vi "Registry.vi"   [LabVIEW 2018, in "GLog.lvlib" / "Registry.lvlib"]
uses:
  Registry.lvlib
  Registry Message.ctl
  Registry Actions.ctl
  api/logger_class/Logger.lvclass
  <vilib>/event_ctls.llb/usereventprio.ctl
  Register Action Data.ctl
  api/logger_class/Logger.lvclass/Logger.ctl
  api/logger_class/Log Record.ctl
  api/logger_class/Internal Log Levels.ctl
  api/logger_class/Log Levels.ctl
  <vilib>/Utility/error.llb/Error Cluster From Error Code.vi
  api/logger_class/Log (Log Record).vi
  <vilib>/ErrorRing/Error Ring.xnode
types:
  T1 = typedef "usereventprio.ctl" = enum32{"high priority", "normal priority"}
  T2 = typedef "GLog.lvlib/Registry.lvlib/Registry Message.ctl" = cluster{"action":T3, "data":variant, "return notifier":refnum<notifier>}
  T3 = typedef "GLog.lvlib/Registry.lvlib/Registry Actions.ctl" = enum16{"Register", "Log", "Enable", "Enable All", "Disable", "Disable All", "Get Enable State", "Get Minimum Log Level", "Set Minimum Log Level", "Set All Minimum Log Level", "Get Logger Info", "Get All Logger Info", "List", "Unregister", "Unregister All", "Shutdown"}
  T4 = typedef "GLog.lvlib/Registry.lvlib/Register Action Data.ctl" = cluster{"Logger":refnum<class "Logger.lvclass">, "Owning VI":string}
  T5 = typedef "GLog.lvlib/Logger.lvclass/Log Record.ctl" = cluster{"level":T6, "timestamp":timestamp, "call chain":string[], "message":string, "data":variant}
  T6 = typedef "GLog.lvlib/Logger.lvclass/Internal Log Levels.ctl" = enum16{"Trace", "Debug", "Info", "Warning", "Error", "Critical", "Internal"}
  T7 = typedef "GLog.lvlib/Logger.lvclass/Log Levels.ctl" = enum16{"Trace", "Debug", "Info", "Warning", "Error", "Critical"}
  T8 = cluster{"logger out":refnum<class "Logger.lvclass">, "error out":errorcluster}
  T9 = cluster{"Enabled?":bool, "error out":errorcluster}
  T10 = cluster{"minimum log level":T7, "error out":errorcluster}
  T11 = cluster{"log level":T7, "error out":errorcluster}
  T12 = cluster{"name":string, "minimum log level":T7, "Enabled?":bool, "error out":errorcluster}
  T13 = cluster{"name":string, "minimum log level":T7, "Enabled?":bool}
  T14 = enum32{"Bad", "Idle", "Run top level", "Running"}[]
  T15 = enum32{"Bad", "Idle", "Run top level", "Running"}
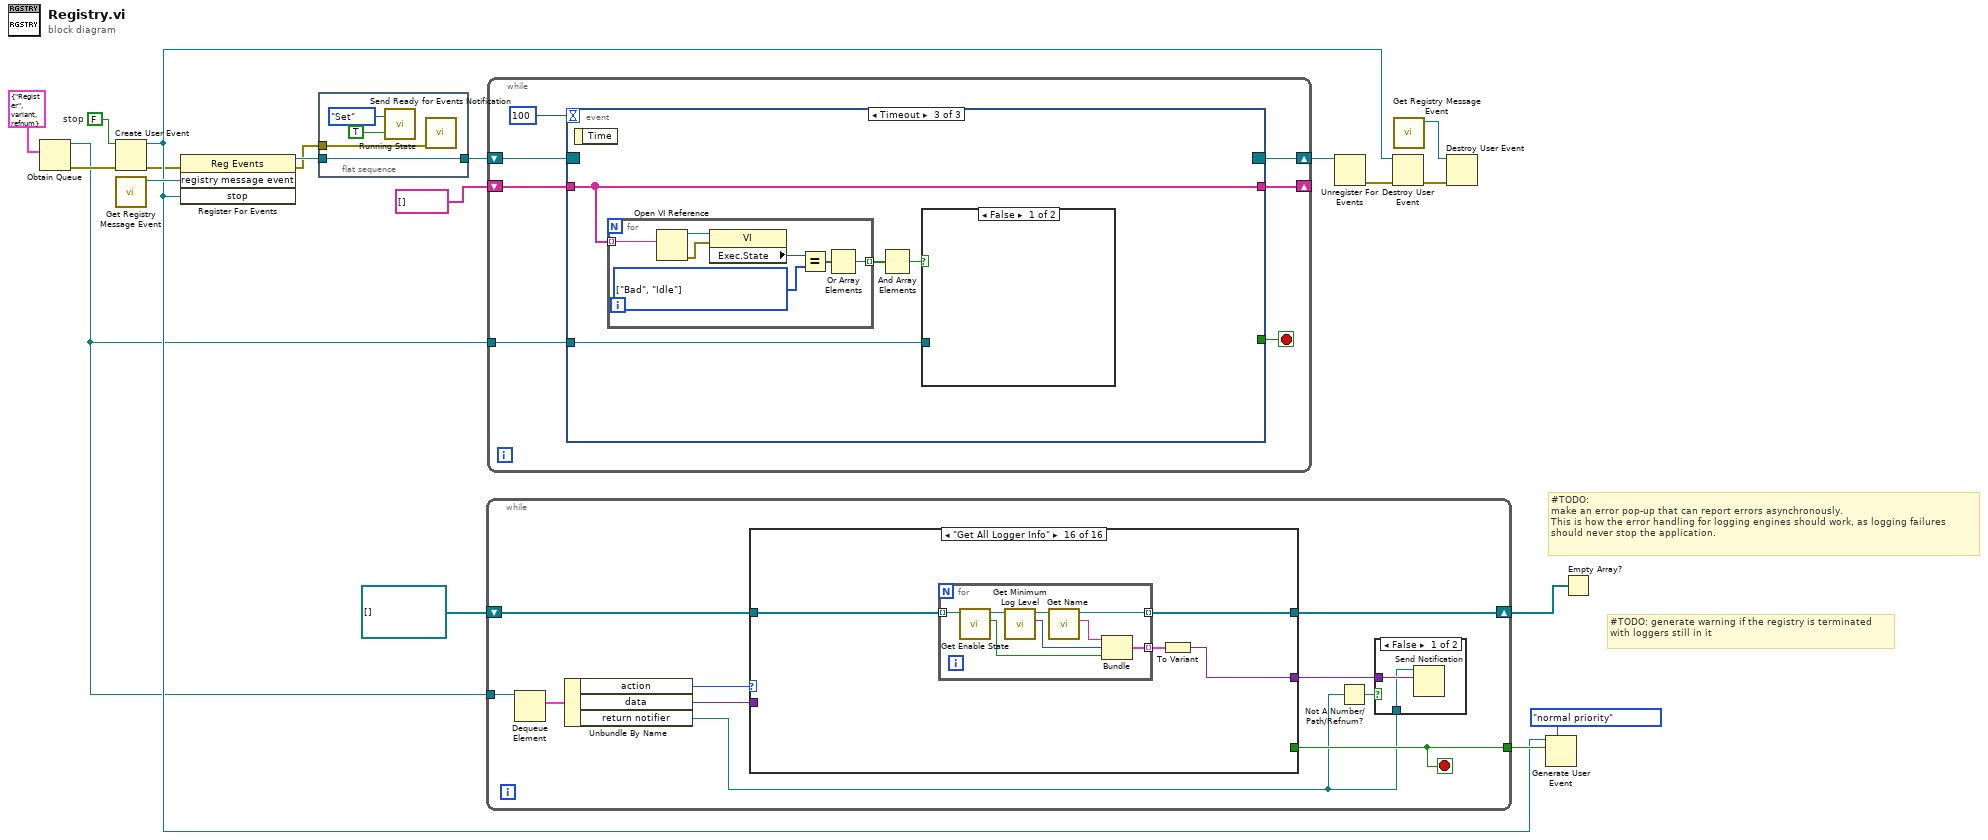
[diagram p0: block diagram]
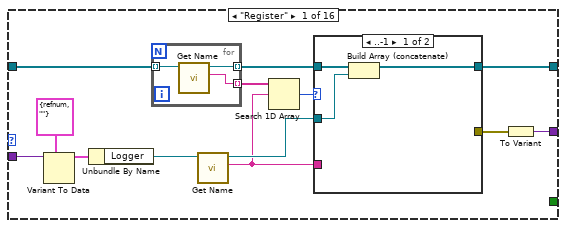
[diagram p2: hidden frame]
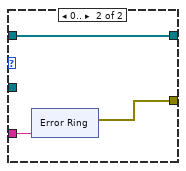
[diagram p3: hidden frame]
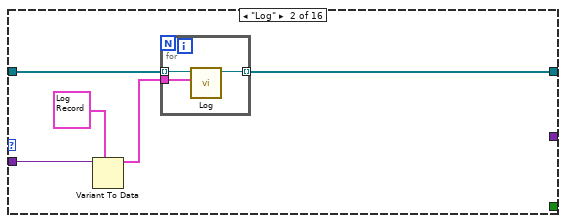
[diagram p4: hidden frame]
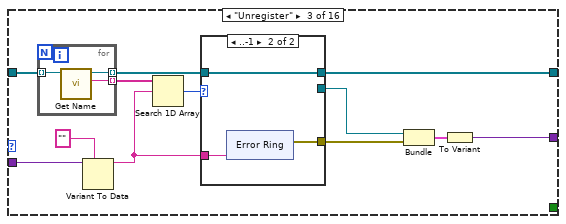
[diagram p5: hidden frame]
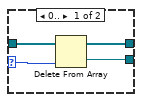
[diagram p6: hidden frame]
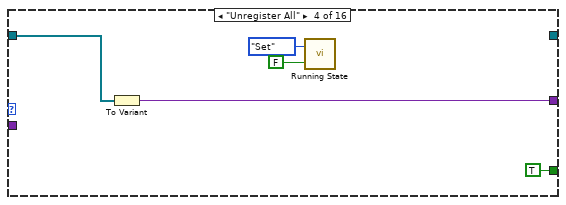
[diagram p7: hidden frame]
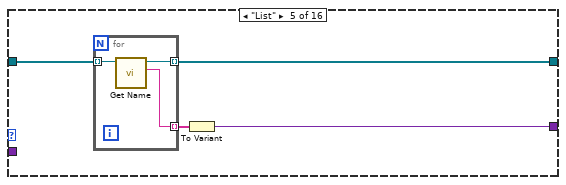
[diagram p8: hidden frame]
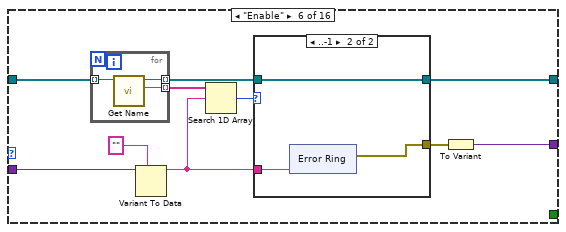
[diagram p9: hidden frame]
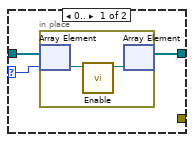
[diagram p10: hidden frame]
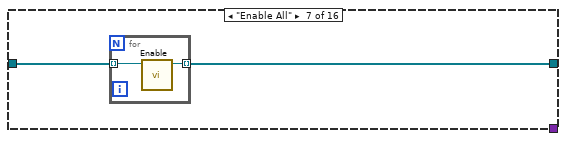
[diagram p11: hidden frame]
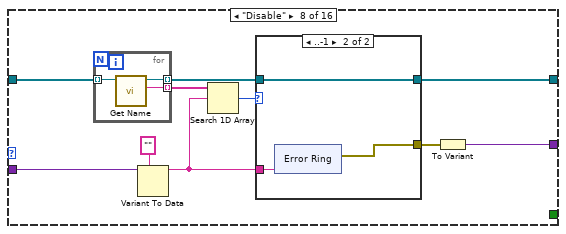
[diagram p12: hidden frame]
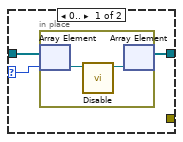
[diagram p13: hidden frame]
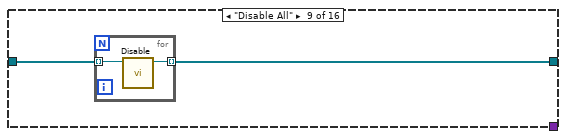
[diagram p14: hidden frame]
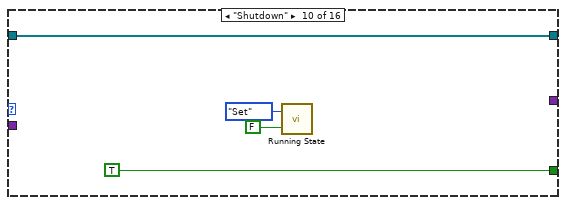
[diagram p15: hidden frame]
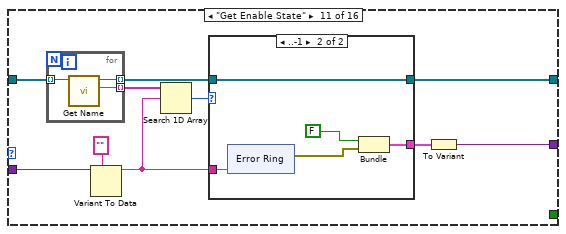
[diagram p16: hidden frame]
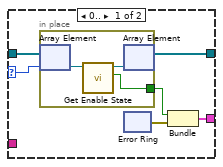
[diagram p17: hidden frame]
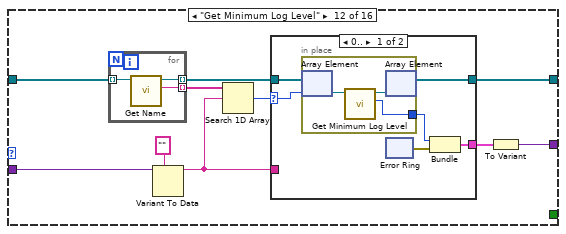
[diagram p18: hidden frame]
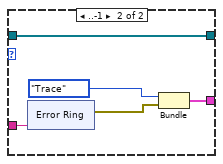
[diagram p19: hidden frame]
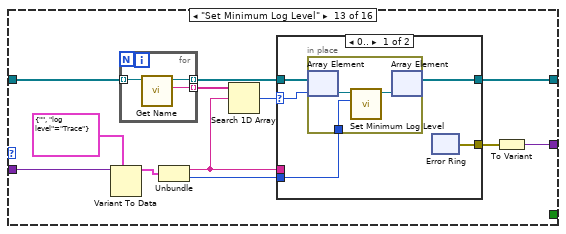
[diagram p20: hidden frame]
diagram:
  w16 = FALSE  # stop
  # "#TODO: generate warning if the registry is terminated with loggers still in it"
  # "#TODO:\nmake an error pop-up that can report errors asynchronously.\nThis is how the error handling for logging engines should work, as logging failures should never stop the application."
  n1 = Obtain Queue(element data type=T2 {"action"=enum."Register", "data"=variant, "return notifier"=refnum} ("registry message")) -> (queue out=w8:refnum<queue>, error out=w10:errorcluster)  [unwired: 4 in, 1 out]
  n2 = Create User Event(user event datatype=w16, error in=w10) -> (user event=w11:refnum<user-event>, error out=w9:errorcluster)
  n3 = call "Get Registry Message Event.vi"() -> ("registry message event"=w13:refnum<user-event>)  [unwired: 11 in]
  n4 = register-events(error in=w9, w13, w11) -> (reference out=w2:refnum<event-registration>, error out=w1:errorcluster)  [unwired: 1 in]
  n5 = flat-sequence {
    tunnel: [w21] -> w3
    tunnel: w2 -> [w21]
    tunnel: w1 -> [w20]
    frame #0 {
      n6 = call "Running State.vi"("value in (F)"=TRUE, "action (get)"=enum16{"Set", "Get"}."Set") -> ()  [unwired: 1 out]
      n7 = call "Send Ready for Events Notification.vi"("error in (no error)"=w20) -> ()  [unwired: 10 in, 1 out]
    }
  }
  n8 = while {
    shift-right: [w24] -> w5
    shift-left: refnum<class "Logger.lvclass">[] [] -> [w33]
    tunnel: w8 -> [w32]
    tunnel: [w28] -> w15
    stop <- w28 stop-if-true
    n9 = Dequeue Element(queue=w32) -> (element=w30:T2)  [unwired: 2 in, 3 out]
    n10 = Unbundle By Name(w30) -> ("action"=w31:T3, "data"=w29:variant, "return notifier"=w25:refnum<notifier>)
    n11 = case shown="\"Get All Logger Info\"" w31 {
      tunnel: w29 -> [w46 w66 w81 _ _ w114 _ w147 _ _ w181 w217 w255 w288 w294 _]
      tunnel: [w44 w64 w72 _ w107 w115 w140 w146 w172 w179 w182 w216 w251 w284 w293 w335] -> w24
      tunnel: w33 -> [w42 w67 w82 w104 w108 w116 w141 w148 w173 w179 w183 w218 w256 w285 w295 w334]
      tunnel: [w35 _ w73 w103 w105 w112 _ w144 _ _ w180 w215 w252 _ w292 w332] -> w27
      tunnel: [_ _ _ TRUE _ _ _ _ _ TRUE _ _ _ _ _ _] -> w28
      frame "Register" {
        n12 = Variant To Data(type=T4 {"Logger"=refnum, "Owning VI"=""} ("Logging.lvlib:Logger.lvclass"), Variant=w46) -> (data=w40:T4)  [unwired: 1 in, 1 out]
        n13 = Unbundle By Name(w40) -> ("Logger"=w34:refnum<class "Logger.lvclass">)
        n14 = for {
          tunnel: w42 -> [w62] mode=indexing
          tunnel: [w61] -> w43 mode=indexing
          tunnel: [w60] -> w41 mode=indexing
          n15 = call "Get Name.vi"("logger in"=w62) -> ("name"=w60:string, "logger out"=w61:refnum<class "Logger.lvclass">)  [unwired: 9 in]
        }
        n16 = call "Get Name.vi"("logger in"=w34) -> ("name"=w37:string, "logger out"=w39:refnum<class "Logger.lvclass">)  [unwired: 9 in]
        n17 = Search 1D Array(1D array=w41, element=w37) -> (index of element=w38:i32)  [unwired: 1 in]
        n18 = case shown="..-1" w38 {
          tunnel: [w49 w52] -> w44
          tunnel: w43 -> [w48 w52]
          tunnel: w39 -> [w47 _]
          tunnel: w37 -> [_ w51]
          tunnel: [_ w50] -> w36
          frame ..-1 {
            n19 = Build Array (concatenate)(w48, w47) -> (w49:refnum<class "Logger.lvclass">[])
          }
          frame 0.. {
            n20 = xnode "Error Ring"("parameter 0"=w51) -> ("error out"=w50:errorcluster)
          }
        }
        n21 = To Variant(anything=w36) -> (Variant=w35:variant)
      }
      frame "Log" {
        n22 = Variant To Data(type=T5 {"level"=enum."Trace", "timestamp"=timestamp(0 s since 1904-01-01), "call chain"=[], "message"="", "data"=variant} ("log record"), Variant=w66) -> (data=w65:T5)  [unwired: 1 in, 1 out]
        n23 = for {
          tunnel: w67 -> [w70] mode=indexing
          tunnel: w65 -> [w68]
          tunnel: [w69] -> w64 mode=indexing
          n24 = call-poly "Log.vi"("log record"=w68, "logger in"=w70) -> ("logger out"=w69:refnum<class "Logger.lvclass">)  [unwired: 9 in]
        }
      }
      frame "Unregister" {
        n25 = for {
          tunnel: w82 -> [w99] mode=indexing
          tunnel: [w98] -> w79 mode=indexing
          tunnel: [w97] -> w77 mode=indexing
          n26 = call "Get Name.vi"("logger in"=w99) -> ("name"=w98:string, "logger out"=w97:refnum<class "Logger.lvclass">)  [unwired: 9 in]
        }
        n27 = Variant To Data(type="", Variant=w81) -> (data=w76:string)  [unwired: 1 in, 1 out]
        n28 = Search 1D Array(1D array=w79, element=w76) -> (index of element=w78:i32)  [unwired: 1 in]
        n29 = case shown="..-1" w78 {
          selector: w78 -> [w85 _]
          tunnel: w77 -> [w86 w89]
          tunnel: [w84 w89] -> w72
          tunnel: w76 -> [_ w88]
          tunnel: [w83 _] -> w75
          tunnel: [_ w87] -> w71
          frame 0.. {
            n30 = Delete From Array(array=w86, index=w85) -> (deleted portion=w83:refnum<class "Logger.lvclass">, array with subset deleted=w84:refnum<class "Logger.lvclass">[])  [unwired: 1 in]
          }
          frame ..-1 {
            n31 = xnode "Error Ring"("parameter 0"=w88) -> ("error out"=w87:errorcluster)
          }
        }
        n32 = Bundle("logger out"=w75, "error out"=w71) -> (w74:T8)  [unwired: 1 in]
        n33 = To Variant(anything=w74) -> (Variant=w73:variant)
      }
      frame "Unregister All" {
        n34 = To Variant(anything=w104) -> (Variant=w103:variant)
        n35 = call "Running State.vi"("value in (F)"=FALSE, "action (get)"=enum16{"Set", "Get"}."Set") -> ()  [unwired: 1 out]
      }
      frame "List" {
        n36 = for {
          tunnel: w108 -> [w111] mode=indexing
          tunnel: [w110] -> w107 mode=indexing
          tunnel: [w109] -> w106 mode=indexing
          n37 = call "Get Name.vi"("logger in"=w111) -> ("name"=w109:string, "logger out"=w110:refnum<class "Logger.lvclass">)  [unwired: 9 in]
        }
        n38 = To Variant(anything=w106) -> (Variant=w105:variant)
      }
      frame "Enable" {
        n39 = for {
          tunnel: w116 -> [w139] mode=indexing
          tunnel: [w138] -> w120 mode=indexing
          tunnel: [w137] -> w118 mode=indexing
          n40 = call "Get Name.vi"("logger in"=w139) -> ("name"=w138:string, "logger out"=w137:refnum<class "Logger.lvclass">)  [unwired: 9 in]
        }
        n41 = Variant To Data(type="", Variant=w114) -> (data=w117:string)  [unwired: 1 in, 1 out]
        n42 = Search 1D Array(1D array=w120, element=w117) -> (index of element=w119:i32)  [unwired: 1 in]
        n43 = case shown="..-1" w119 {
          selector: w119 -> [w123 _]
          tunnel: w118 -> [w124 w129]
          tunnel: [w122 w129] -> w115
          tunnel: w117 -> [_ w128]
          tunnel: [_ w127] -> w113
          frame 0.. {
            n44 = in-place {
              n45 = in-place-array #1(w124, w123) -> (w126:refnum<class "Logger.lvclass">)
              n46 = call "Enable.vi"("logger in"=w126) -> ("logger out"=w125:refnum<class "Logger.lvclass">)  [unwired: 10 in]
              n47 = in-place-array #1(w125) -> (w122:refnum<class "Logger.lvclass">[])  [unwired: 1 out]
            }
          }
          frame ..-1 {
            n48 = xnode "Error Ring"("parameter 0"=w128) -> ("error out"=w127:errorcluster)
          }
        }
        n49 = To Variant(anything=w113) -> (Variant=w112:variant)
      }
      frame "Enable All" {
        n50 = for {
          tunnel: w141 -> [w143] mode=indexing
          tunnel: [w142] -> w140 mode=indexing
          n51 = call "Enable.vi"("logger in"=w143) -> ("logger out"=w142:refnum<class "Logger.lvclass">)  [unwired: 10 in]
        }
      }
      frame "Disable" {
        n52 = for {
          tunnel: w148 -> [w171] mode=indexing
          tunnel: [w170] -> w152 mode=indexing
          tunnel: [w169] -> w150 mode=indexing
          n53 = call "Get Name.vi"("logger in"=w171) -> ("name"=w170:string, "logger out"=w169:refnum<class "Logger.lvclass">)  [unwired: 9 in]
        }
        n54 = Variant To Data(type="", Variant=w147) -> (data=w149:string)  [unwired: 1 in, 1 out]
        n55 = Search 1D Array(1D array=w152, element=w149) -> (index of element=w151:i32)  [unwired: 1 in]
        n56 = case shown="..-1" w151 {
          selector: w151 -> [w155 _]
          tunnel: w150 -> [w156 w161]
          tunnel: [w154 w161] -> w146
          tunnel: w149 -> [_ w160]
          tunnel: [_ w159] -> w145
          frame 0.. {
            n57 = in-place {
              n58 = in-place-array #2(w156, w155) -> (w158:refnum<class "Logger.lvclass">)
              n59 = call "Disable.vi"("logger in"=w158) -> ("logger out"=w157:refnum<class "Logger.lvclass">)  [unwired: 10 in]
              n60 = in-place-array #2(w157) -> (w154:refnum<class "Logger.lvclass">[])  [unwired: 1 out]
            }
          }
          frame ..-1 {
            n61 = xnode "Error Ring"("parameter 0"=w160) -> ("error out"=w159:errorcluster)
          }
        }
        n62 = To Variant(anything=w145) -> (Variant=w144:variant)
      }
      frame "Disable All" {
        n63 = for {
          tunnel: w173 -> [w175] mode=indexing
          tunnel: [w174] -> w172 mode=indexing
          n64 = call "Disable.vi"("logger in"=w175) -> ("logger out"=w174:refnum<class "Logger.lvclass">)  [unwired: 10 in]
        }
      }
      frame "Shutdown" {
        n65 = call "Running State.vi"("value in (F)"=FALSE, "action (get)"=enum16{"Set", "Get"}."Set") -> ()  [unwired: 1 out]
      }
      frame "Get Enable State" {
        n66 = for {
          tunnel: w183 -> [w214] mode=indexing
          tunnel: [w213] -> w188 mode=indexing
          tunnel: [w212] -> w186 mode=indexing
          n67 = call "Get Name.vi"("logger in"=w214) -> ("name"=w213:string, "logger out"=w212:refnum<class "Logger.lvclass">)  [unwired: 9 in]
        }
        n68 = Variant To Data(type="", Variant=w181) -> (data=w185:string)  [unwired: 1 in, 1 out]
        n69 = Search 1D Array(1D array=w188, element=w185) -> (index of element=w187:i32)  [unwired: 1 in]
        n70 = case shown="..-1" w187 {
          selector: w187 -> [w194 _]
          tunnel: w186 -> [w195 w204]
          tunnel: [w193 w204] -> w182
          tunnel: w185 -> [_ w203]
          tunnel: [w191 w201] -> w184
          frame 0.. {
            n71 = in-place {
              in-place-border: [w197] -> w192
              n72 = in-place-array #3(w195, w194) -> (w199:refnum<class "Logger.lvclass">)
              n73 = call "Get Enable State.vi"("logger in"=w199) -> ("Enabled?"=w197:bool, "logger out"=w198:refnum<class "Logger.lvclass">)  [unwired: 9 in]
              n74 = in-place-array #3(w198) -> (w193:refnum<class "Logger.lvclass">[])  [unwired: 1 out]
            }
            n75 = xnode "Error Ring"() -> ("error out"=w190:errorcluster)
            n76 = Bundle("Enabled?"=w192, "error out"=w190) -> (w191:T9)  [unwired: 1 in]
          }
          frame ..-1 {
            n77 = xnode "Error Ring"("parameter 0"=w203) -> ("error out"=w202:errorcluster)
            n78 = Bundle(FALSE, "error out"=w202) -> (w201:cluster{bool, "error out":errorcluster})  [unwired: 1 in]
          }
        }
        n79 = To Variant(anything=w184) -> (Variant=w180:variant)
      }
      frame "Get Minimum Log Level" {
        n80 = for {
          tunnel: w218 -> [w249] mode=indexing
          tunnel: [w248] -> w223 mode=indexing
          tunnel: [w247] -> w221 mode=indexing
          n81 = call "Get Name.vi"("logger in"=w249) -> ("name"=w248:string, "logger out"=w247:refnum<class "Logger.lvclass">)  [unwired: 9 in]
        }
        n82 = Variant To Data(type="", Variant=w217) -> (data=w220:string)  [unwired: 1 in, 1 out]
        n83 = Search 1D Array(1D array=w223, element=w220) -> (index of element=w222:i32)  [unwired: 1 in]
        n84 = case shown="0.." w222 {
          selector: w222 -> [w229 _]
          tunnel: w221 -> [w230 w239]
          tunnel: [w228 w239] -> w216
          tunnel: w220 -> [_ w238]
          tunnel: [w226 w236] -> w219
          frame 0.. {
            n85 = in-place {
              in-place-border: [w232] -> w227
              n86 = in-place-array #4(w230, w229) -> (w234:refnum<class "Logger.lvclass">)
              n87 = call "Get Minimum Log Level.vi"("logger in"=w234) -> ("minimum log level"=w232:T7, "logger out"=w233:refnum<class "Logger.lvclass">)  [unwired: 9 in]
              n88 = in-place-array #4(w233) -> (w228:refnum<class "Logger.lvclass">[])  [unwired: 1 out]
            }
            n89 = xnode "Error Ring"() -> ("error out"=w225:errorcluster)
            n90 = Bundle("minimum log level"=w227, "error out"=w225) -> (w226:T10)  [unwired: 1 in]
          }
          frame ..-1 {
            n91 = xnode "Error Ring"("parameter 0"=w238) -> ("error out"=w237:errorcluster)
            n92 = Bundle("log level"=Log_Levels."Trace", "error out"=w237) -> (w236:T11)  [unwired: 1 in]
          }
        }
        n93 = To Variant(anything=w219) -> (Variant=w215:variant)
      }
      frame "Set Minimum Log Level" {
        n94 = Variant To Data(type=cluster{string, "log level":T7} {"", "log level"=enum."Trace"}, Variant=w255) -> (data=w258:cluster{string, "log level":T7})  [unwired: 1 in, 1 out]
        n95 = for {
          tunnel: w256 -> [w283] mode=indexing
          tunnel: [w282] -> w261 mode=indexing
          tunnel: [w281] -> w259 mode=indexing
          n96 = call "Get Name.vi"("logger in"=w283) -> ("name"=w282:string, "logger out"=w281:refnum<class "Logger.lvclass">)  [unwired: 9 in]
        }
        n97 = Unbundle(w258) -> (w253:string, "log level"=w250:T7)
        n98 = Search 1D Array(1D array=w261, element=w253) -> (index of element=w260:i32)  [unwired: 1 in]
        n99 = case shown="0.." w260 {
          selector: w260 -> [w265 _]
          tunnel: w259 -> [w266 w273]
          tunnel: [w264 w273] -> w251
          tunnel: w253 -> [_ w272]
          tunnel: [w263 w271] -> w257
          tunnel: w250 -> [w262 _]
          frame 0.. {
            n100 = in-place {
              in-place-border: w262 -> [w268]
              n101 = in-place-array #5(w266, w265) -> (w270:refnum<class "Logger.lvclass">)
              n102 = call "Set Minimum Log Level.vi"("minimum log level"=w268, "logger in"=w270) -> ("logger out"=w269:refnum<class "Logger.lvclass">)  [unwired: 9 in]
              n103 = in-place-array #5(w269) -> (w264:refnum<class "Logger.lvclass">[])  [unwired: 1 out]
            }
            n104 = xnode "Error Ring"() -> ("error out"=w263:errorcluster)
          }
          frame ..-1 {
            n105 = xnode "Error Ring"("parameter 0"=w272) -> ("error out"=w271:errorcluster)
          }
        }
        n106 = To Variant(anything=w257) -> (Variant=w252:variant)
      }
      frame "Set All Minimum Log Level" {
        n107 = Variant To Data(type=Log_Levels."Trace" ("log level"), Variant=w288) -> (data=w286:T7)  [unwired: 1 in, 1 out]
        n108 = for {
          tunnel: w285 -> [w291] mode=indexing
          tunnel: [w290] -> w284 mode=indexing
          tunnel: w286 -> [w289]
          n109 = call "Set Minimum Log Level.vi"("minimum log level"=w289, "logger in"=w291) -> ("logger out"=w290:refnum<class "Logger.lvclass">)  [unwired: 9 in]
        }
      }
      frame "Get Logger Info" {
        n110 = for {
          tunnel: w295 -> [w331] mode=indexing
          tunnel: [w330] -> w300 mode=indexing
          tunnel: [w329] -> w298 mode=indexing
          n111 = call "Get Name.vi"("logger in"=w331) -> ("name"=w330:string, "logger out"=w329:refnum<class "Logger.lvclass">)  [unwired: 9 in]
        }
        n112 = Variant To Data(type="", Variant=w294) -> (data=w297:string)  [unwired: 1 in, 1 out]
        n113 = Search 1D Array(1D array=w300, element=w297) -> (index of element=w299:i32)  [unwired: 1 in]
        n114 = case shown="0.." w299 {
          selector: w299 -> [w308 _]
          tunnel: w298 -> [w309 w321]
          tunnel: [w307 w321] -> w293
          tunnel: w297 -> [_ w320]
          tunnel: [w305 _] -> w296
          frame 0.. {
            n115 = in-place {
              in-place-border: [w315] -> w306
              in-place-border: [w312] -> w303
              in-place-border: [w311] -> w302
              n116 = in-place-array #6(w309, w308) -> (w317:refnum<class "Logger.lvclass">)
              n117 = call "Get Enable State.vi"("logger in"=w317) -> ("Enabled?"=w315:bool, "logger out"=w316:refnum<class "Logger.lvclass">)  [unwired: 9 in]
              n118 = call "Get Minimum Log Level.vi"("logger in"=w316) -> ("minimum log level"=w312:T7, "logger out"=w314:refnum<class "Logger.lvclass">)  [unwired: 9 in]
              n119 = call "Get Name.vi"("logger in"=w314) -> ("name"=w311:string, "logger out"=w313:refnum<class "Logger.lvclass">)  [unwired: 9 in]
              n120 = in-place-array #6(w313) -> (w307:refnum<class "Logger.lvclass">[])  [unwired: 1 out]
            }
            n121 = xnode "Error Ring"() -> ("error out"=w304:errorcluster)
            n122 = Bundle("name"=w302, "minimum log level"=w303, "Enabled?"=w306, "error out"=w304) -> (w305:T12)  [unwired: 1 in]
          }
          frame ..-1 {
            n123 = xnode "Error Ring"("parameter 0"=w320) -> ("error out"=w319:errorcluster)
            n124 = Bundle(FALSE, "error out"=w319) -> ()  [unwired: 1 in, 1 out]
          }
        }
        n125 = To Variant(anything=w296) -> (Variant=w292:variant)
      }
      frame "Get All Logger Info" {
        n126 = for {
          tunnel: [w338] -> w335 mode=indexing
          tunnel: w334 -> [w337] mode=indexing
          tunnel: [w336] -> w333 mode=indexing
          n127 = call "Get Enable State.vi"("logger in"=w337) -> ("Enabled?"=w343:bool, "logger out"=w340:refnum<class "Logger.lvclass">)  [unwired: 9 in]
          n128 = call "Get Minimum Log Level.vi"("logger in"=w340) -> ("minimum log level"=w342:T7, "logger out"=w339:refnum<class "Logger.lvclass">)  [unwired: 9 in]
          n129 = call "Get Name.vi"("logger in"=w339) -> ("name"=w341:string, "logger out"=w338:refnum<class "Logger.lvclass">)  [unwired: 9 in]
          n130 = Bundle("name"=w341, "minimum log level"=w342, "Enabled?"=w343) -> (w336:T13)  [unwired: 1 in]
        }
        n131 = To Variant(anything=w333) -> (Variant=w332:variant)
      }
    }
    n132 = Not A Number/Path/Refnum?(number/path/refnum=w25) -> (NaN/Path/Refnum?=w26:bool)
    n133 = case shown="False" w26 {
      tunnel: w25 -> [w344 _]
      tunnel: w27 -> [w345 _]
      frame False {
        n134 = Send Notification(notification=w345, notifier=w344) -> ()  [unwired: 1 in, 2 out]
      }
      frame True {
      }
    }
  }
  n135 = while {
    tunnel: w8 -> [w352]
    shift-right: [w350] -> w17
    shift-left: w3 -> [w349]
    shift-right: [w346] -> _
    shift-left: string[] [] ("1D array") -> [w347]
    stop <- w348 stop-if-true
    n136 = event shown="[2] Timeout" {
      selector: w349 -> [_ _ _]
      dyn-events: [_ _ _] -> w350
      timeout: 100 -> [_ _ _]
      tunnel: w352 -> [w358 _ w379]
      tunnel: [_ w375 _] -> w348
      tunnel: w347 -> [w354 w374 w378]
      tunnel: [w355 w374 w378] -> w346
      event User Event {
        n137 = event-data() -> ("action"=w353:T3, "data"=w356:variant, "return notifier"=w357:refnum<notifier>)  [unwired: 1 in]
        n138 = Bundle By Name(cluster=T2 {"action"=enum."Register", "data"=variant, "return notifier"=refnum} ("registry message"), "action"=w353, "data"=w356, "return notifier"=w357) -> (w359:T2)
        n139 = case shown="Default" w353 {
          tunnel: w356 -> [w366 _]
          tunnel: [w363 w373] -> w355
          tunnel: w354 -> [w361 w373]
          frame "Register" {
            n140 = Variant To Data(type=T4 {"Logger"=refnum, "Owning VI"=""} ("Logging.lvlib:Logger.lvclass"), Variant=w366) -> (data=w367:T4)  [unwired: 1 in, 1 out]
            n141 = Unbundle By Name(w367) -> ("Owning VI"=w364:string)
            n142 = Search 1D Array(1D array=w361, element=w364) -> (index of element=w365:i32)  [unwired: 1 in]
            n143 = Less Than 0?(x=w365) -> (x < 0?=w362:bool)
            n144 = case shown="False" w362 {
              tunnel: w361 -> [w369 w372]
              tunnel: w364 -> [_ w371]
              tunnel: [w369 w370] -> w363
              frame False {
              }
              frame True {
                n145 = Build Array (concatenate)(w372, w371) -> (w370:string[])
              }
            }
          }
          frame Default {
          }
        }
        n146 = Enqueue Element(queue=w358, element=w359) -> ()  [unwired: 2 in, 3 out]
      }
      event User Event {
        n147 = event-data() -> ("stop"=w375:bool)  [unwired: 1 in]
      }
      event Timeout {
        n148 = event-data() -> ()  [unwired: 1 in, 1 out]
        n149 = for {
          tunnel: w378 -> [w386] mode=indexing
          tunnel: [w380] -> w377 mode=indexing
          w383 = T14 [enum."Bad", enum."Idle"] items=["Bad", "Idle", "Run top level", "Running"] ("Execution:State")
          n150 = Open VI Reference(vi path=w386) -> (vi reference=w385:refnum<vi>, error out=w381:errorcluster)  [unwired: 5 in]
          n151 = property class="VI"(reference=w385, error in=w381) -> ("Exec.State"=w384:T15)  [unwired: 2 out]
          n152 = Equal?(x=w384, y=w383) -> (x = y?=w382:bool[])
          n153 = Or Array Elements(Boolean array=w382) -> (logical OR=w380:bool)
        }
        n154 = And Array Elements(Boolean array=w377) -> (logical AND=w376:bool)
        n155 = case shown="False" w376 {
          tunnel: w379 -> [_ w388]
          frame False {
          }
          frame True {
            n156 = Enqueue Element(queue=w388, element=T2 {"action"=enum."Shutdown", "data"=variant, "return notifier"=refnum} ("registry message")) -> ()  [unwired: 2 in, 3 out]
          }
        }
      }
    }
  }
  n157 = Unregister For Events(event registration refnum=w17) -> (error out=w7:errorcluster)  [unwired: 1 in]
  n158 = Destroy User Event(user event=w11, error in=w7) -> (error out=w6:errorcluster)
  n159 = call "Get Registry Message Event.vi"() -> ("registry message event"=w12:refnum<user-event>)  [unwired: 11 in]
  n160 = Destroy User Event(user event=w12, error in=w6) -> ()  [unwired: 1 out]
  n161 = Generate User Event(priority (normal)=usereventprio."normal priority", user event=w11, event data cluster=w15) -> ()  [unwired: 1 in, 2 out]
  n162 = Empty Array?(array=w5) -> ()  [unwired: 1 out]
